vi "test tools list output schema.vi"(8 "error in (no error)":errorcluster) -> (0 "error out":errorcluster, 3 "body":string)   [LabVIEW 2020, in "MCP Server tests.lvlib"]
doc: "tools/list gives every tool with non-picture outputs an outputSchema. For fake_tool_picture_outputs it is an object schema whose properties and required list exactly count, label, mode and time, the names that tools/call returns in structuredContent, without the picture output. The property schemas are built like the input schemas, without default: time (timestamp) is a string with format date-time, mode (enum) has enum [\"slow\",\"fast\"], count is an integer with the description of its indicator. A tool without outputs (fake_tool_no_inputs_outputs) has no outputSchema. The requests are sent with the LabVIEW HTTP Client directly."
uses:
  MCP Server tests.lvlib
  76897956-0dee-4ca4-8c48-61d2eaeac07d.vi
  c19c7c96-80ec-4cdf-8c59-ab371bb35518.vi
  31ad5ed3-fed4-46a9-ac69-80efe7dec1a8.vi
  8415a791-681a-46d9-8f15-2bdb6ca1e76c.vi
  <vilib>/JDP Science/JSONtext/Next JSON Value.vi
  <vilib>/JDP Science/JSONtext/String Subset.vi
  <vilib>/JDP Science/JSONtext/Parsing/Advance past next JSON Value (inlined COPY).vi
  <vilib>/JDP Science/JSONtext/Parsing/Advance past whitespace.vi
  <vilib>/JDP Science/JSONtext/Parsing/Advance past String.vi
  <vilib>/JDP Science/JSONtext/Parsing/Advance past Number.vi
  <vilib>/JDP Science/JSONtext/Parsing/Advance past Line Ending.vi
  <vilib>/JDP Science/JSONtext/Parsing/Parse Full Path or Item Name.vi
  <vilib>/JDP Science/JSONtext/Parsing/Advance past Array.vi
  <vilib>/JDP Science/JSONtext/Parsing/Advance past Object.vi
  <vilib>/JDP Science/JSONtext/support/Error Cluster From Code.vi
  <vilib>/JDP Science/JSONtext/Offset/Find Item Locations by Path.vi
  <vilib>/JDP Science/JSONtext/JSON text to Variant.vi
  <vilib>/JDP Science/JSONtext/LVClass Serializer/JSONtext LVClass Serializer.lvclass
  <vilib>/addons/_JKI Toolkits/Caraya/classes/Test/Test.lvclass
  <vilib>/JDP Science/JSONtext/JSONtext.lvlib
  <vilib>/addons/_JKI Toolkits/Caraya/classes/Assert/Assert.lvclass
panel:
  out "lookup error":errorcluster
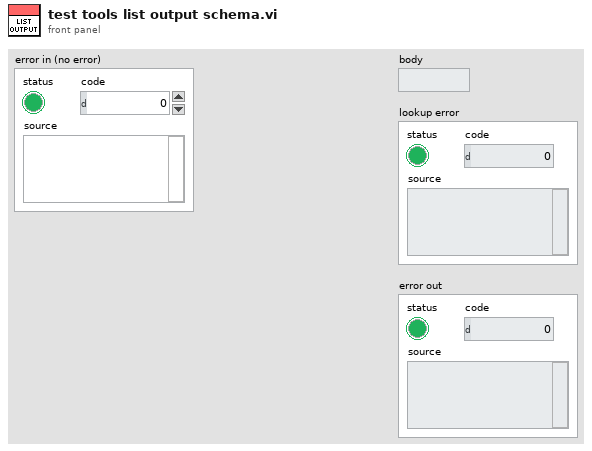
[diagram p1: front panel]
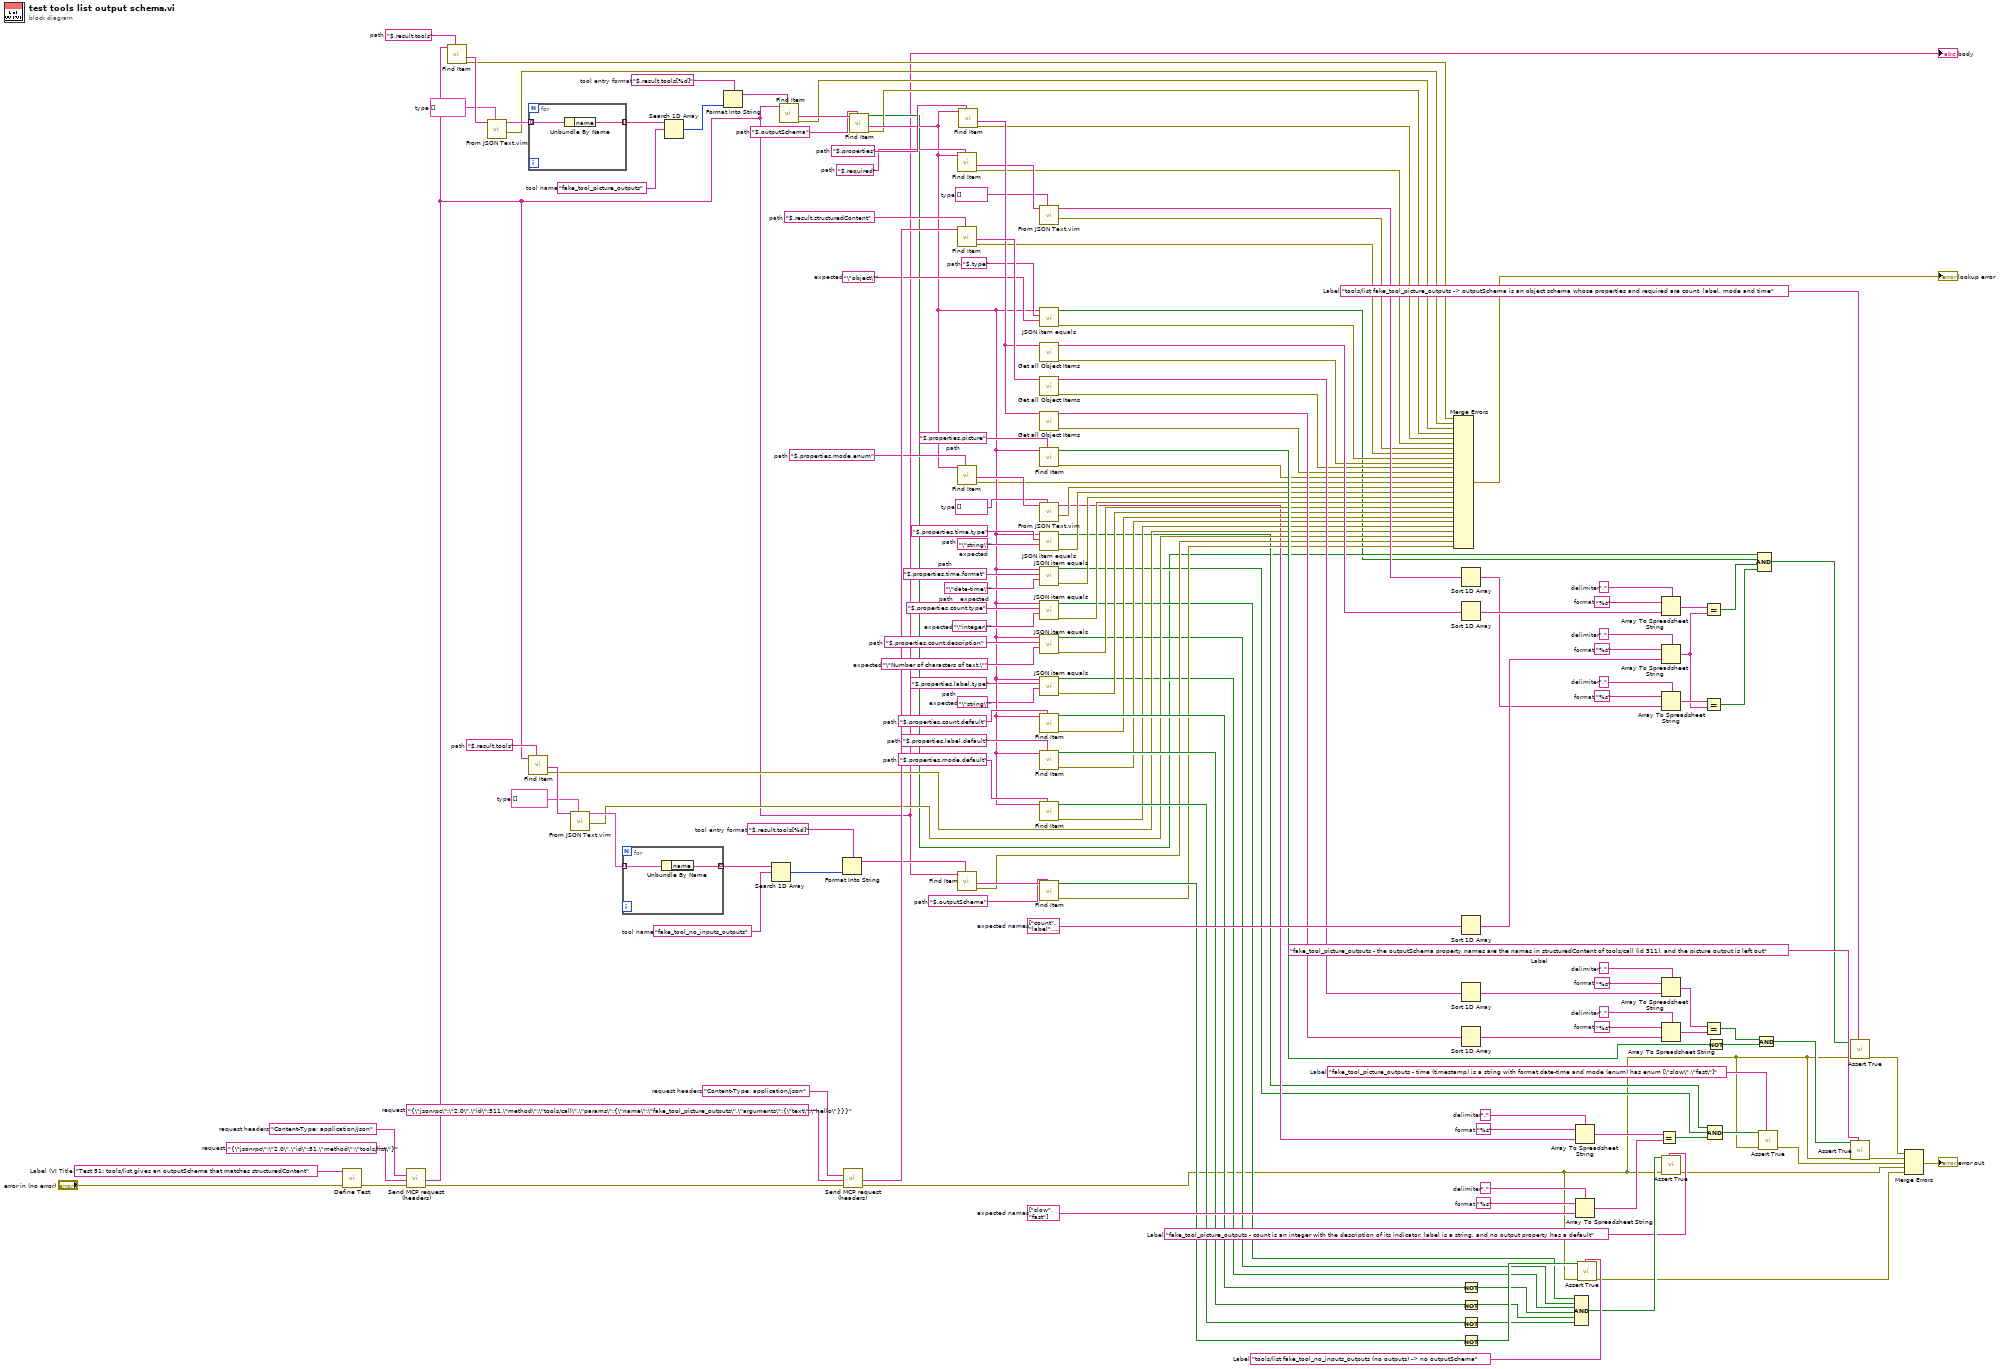
[diagram p0: block diagram]
diagram:
  w143 = "Content-Type: application/json"  # request headers
  w148 = "Content-Type: application/json"  # request headers
  w82 = "tools/list fake_tool_no_inputs_outputs (no outputs) -> no outputSchema"  # Label
  w30 = "fake_tool_picture_outputs - count is an integer with the description of its indicator, label is a string, and no output property has a default"  # Label
  w14 = "fake_tool_picture_outputs - time (timestamp) is a string with format date-time and mode (enum) has enum [\"slow\",\"fast\"]"  # Label
  w12 = "fake_tool_picture_outputs - the outputSchema property names are the names in structuredContent of tools/call (id 511), and the picture output is left out"  # Label
  w9 = "tools/list fake_tool_picture_outputs -> outputSchema is an object schema whose properties and required are count, label, mode and time"  # Label
  w114 = "$.outputSchema"  # path
  w123 = "$.result.tools[%d]"  # tool entry format
  w128 = "fake_tool_no_inputs_outputs"  # tool name
  w137 = cluster{"name":string}[] []  # type
  w144 = "$.result.tools"  # path
  w107 = "$.properties.mode.default"  # path
  w108 = "$.properties.label.default"  # path
  w109 = "$.properties.count.default"  # path
  w87 = "\"string\""  # expected
  w88 = "$.properties.label.type"  # path
  w90 = "\"Number of characters of text.\""  # expected
  w91 = "$.properties.count.description"  # path
  w92 = "\"integer\""  # expected
  w93 = "$.properties.count.type"  # path
  w152 = ","  # delimiter
  w154 = "%s"  # format
  w153 = string[] ["slow", "fast"]  # expected names
  w49 = ","  # delimiter
  w51 = "%s"  # format
  w94 = "\"date-time\""  # expected
  w95 = "$.properties.time.format"  # path
  w96 = "\"string\""  # expected
  w97 = "$.properties.time.type"  # path
  w98 = string[] []  # type
  w110 = "$.properties.mode.enum"  # path
  w111 = "$.properties.picture"  # path
  w37 = ","  # delimiter
  w39 = "%s"  # format
  w120 = ","  # delimiter
  w122 = "%s"  # format
  w34 = ","  # delimiter
  w36 = "%s"  # format
  w40 = ","  # delimiter
  w42 = "%s"  # format
  w101 = "\"object\""  # expected
  w102 = "$.type"  # path
  w149 = ","  # delimiter
  w151 = "%s"  # format
  w155 = string[] ["count", "label", "mode", "time"]  # expected names
  w135 = "$.result.structuredContent"  # path
  w103 = string[] []  # type
  w112 = "$.required"  # path
  w113 = "$.properties"  # path
  w116 = "$.outputSchema"  # path
  w125 = "$.result.tools[%d]"  # tool entry format
  w130 = "fake_tool_picture_outputs"  # tool name
  w139 = cluster{"name":string}[] []  # type
  w145 = "$.result.tools"  # path
  w142 = "{\"jsonrpc\":\"2.0\",\"id\":511,\"method\":\"tools/call\",\"params\":{\"name\":\"fake_tool_picture_outputs\",\"arguments\":{\"text\":\"hello\"}}}"  # request
  w147 = "{\"jsonrpc\":\"2.0\",\"id\":51,\"method\":\"tools/list\"}"  # request
  w157 = "Test 51: tools/list gives an outputSchema that matches structuredContent"  # Label (VI Title)
  n1 = call <vilib>:"Define Test.vi"("error in (no error)"="error in (no error)", "Label (VI Title)"=w157) -> ("error out"=w146:errorcluster)  [unwired: 8 in, 1 out]
  n2 = call "Send MCP request (headers).vi"("error in (no error)"=w146, "request"=w147, "request headers"=w148) -> ("error out"=w141:errorcluster, "response"=w3:string)  [unwired: 5 in, 2 out]
  "body" <- w3
  n3 = call <vilib>:"Find Item.vi"("$Path or Item Name"=w145, "JSON"=w3) -> ("error out"=w78:errorcluster, "<JSON>"=w140:string)  [unwired: 6 in, 2 out]
  n4 = call "From JSON Text.vim"("Data Type and Default Value"=w139, "JSON"=w140) -> ("error out"=w77:errorcluster, "Data out"=w134:cluster{"name":string}[])  [unwired: 8 in]
  n5 = for {
    tunnel: w134 -> [w159] mode=indexing
    tunnel: [w158] -> w131 mode=indexing
    n6 = Unbundle By Name(w159) -> ("name"=w158:string)
  }
  n7 = call <vilib>:"Find Item.vi"("$Path or Item Name"=w144, "JSON"=w3) -> ("error out"=w55:errorcluster, "<JSON>"=w138:string)  [unwired: 6 in, 2 out]
  n8 = call "From JSON Text.vim"("Data Type and Default Value"=w137, "JSON"=w138) -> ("error out"=w54:errorcluster, "Data out"=w133:cluster{"name":string}[])  [unwired: 8 in]
  n9 = for {
    tunnel: w133 -> [w161] mode=indexing
    tunnel: [w160] -> w129 mode=indexing
    n10 = Unbundle By Name(w161) -> ("name"=w160:string)
  }
  n11 = Search 1D Array(1D array=w131, element=w130) -> (index of element=w126:i32)  [unwired: 1 in]
  n12 = Format Into String(format string=w125, w126) -> (resulting string=w119:string)  [unwired: 2 in, 1 out]
  n13 = Search 1D Array(1D array=w129, element=w128) -> (index of element=w124:i32)  [unwired: 1 in]
  n14 = call <vilib>:"Find Item.vi"("$Path or Item Name"=w119, "JSON"=w3) -> ("error out"=w76:errorcluster, "<JSON>"=w117:string)  [unwired: 6 in, 2 out]
  n15 = Format Into String(format string=w123, w124) -> (resulting string=w118:string)  [unwired: 2 in, 1 out]
  n16 = call "Send MCP request (headers).vi"("error in (no error)"=w141, "request"=w142, "request headers"=w143) -> ("error out"=w10:errorcluster, "response"=w136:string)  [unwired: 5 in, 2 out]
  n17 = call <vilib>:"Find Item.vi"("$Path or Item Name"=w116, "JSON"=w117) -> ("error out"=w75:errorcluster, "<JSON>"=w89:string, "Found"=w19:bool)  [unwired: 6 in, 1 out]
  n18 = call <vilib>:"Find Item.vi"("$Path or Item Name"=w112, "JSON"=w89) -> ("error out"=w73:errorcluster, "<JSON>"=w104:string)  [unwired: 6 in, 2 out]
  n19 = call <vilib>:"Find Item.vi"("$Path or Item Name"=w135, "JSON"=w136) -> ("error out"=w71:errorcluster, "<JSON>"=w132:string)  [unwired: 6 in, 2 out]
  n20 = call <vilib>:"Find Item.vi"("$Path or Item Name"=w110, "JSON"=w89) -> ("error out"=w65:errorcluster, "<JSON>"=w99:string)  [unwired: 6 in, 2 out]
  n21 = call <vilib>:"Find Item.vi"("$Path or Item Name"=w118, "JSON"=w3) -> ("error out"=w53:errorcluster, "<JSON>"=w115:string)  [unwired: 6 in, 2 out]
  n22 = call <vilib>:"Find Item.vi"("$Path or Item Name"=w113, "JSON"=w89) -> ("error out"=w74:errorcluster, "<JSON>"=w105:string)  [unwired: 6 in, 2 out]
  n23 = call "From JSON Text.vim"("Data Type and Default Value"=w103, "JSON"=w104) -> ("error out"=w72:errorcluster, "Data out"=w79:string[])  [unwired: 8 in]
  n24 = call "JSON item equals.vi"("expected"=w101, "path"=w102, "JSON"=w89) -> ("error out"=w70:errorcluster, "equal?"=w18:bool)  [unwired: 6 in, 1 out]
  n25 = call <vilib>:"Get all Object Items.vi"("JSON"=w105) -> ("error out"=w69:errorcluster, "Item Names"=w81:string[])  [unwired: 7 in, 2 out]
  n26 = call <vilib>:"Get all Object Items.vi"("JSON"=w132) -> ("error out"=w68:errorcluster, "Item Names"=w127:string[])  [unwired: 7 in, 2 out]
  n27 = call <vilib>:"Get all Object Items.vi"("JSON"=w105) -> ("error out"=w67:errorcluster, "Item Names"=w80:string[])  [unwired: 7 in, 2 out]
  n28 = call <vilib>:"Find Item.vi"("$Path or Item Name"=w111, "JSON"=w89) -> ("error out"=w66:errorcluster, "Found"=w100:bool)  [unwired: 6 in, 2 out]
  n29 = call "From JSON Text.vim"("Data Type and Default Value"=w98, "JSON"=w99) -> ("error out"=w64:errorcluster, "Data out"=w50:string[])  [unwired: 8 in]
  n30 = call "JSON item equals.vi"("expected"=w96, "path"=w97, "JSON"=w89) -> ("error out"=w63:errorcluster, "equal?"=w24:bool)  [unwired: 6 in, 1 out]
  n31 = call "JSON item equals.vi"("expected"=w94, "path"=w95, "JSON"=w89) -> ("error out"=w62:errorcluster, "equal?"=w23:bool)  [unwired: 6 in, 1 out]
  n32 = call "JSON item equals.vi"("expected"=w92, "path"=w93, "JSON"=w89) -> ("error out"=w61:errorcluster, "equal?"=w48:bool)  [unwired: 6 in, 1 out]
  n33 = call "JSON item equals.vi"("expected"=w90, "path"=w91, "JSON"=w89) -> ("error out"=w60:errorcluster, "equal?"=w47:bool)  [unwired: 6 in, 1 out]
  n34 = call "JSON item equals.vi"("expected"=w87, "path"=w88, "JSON"=w89) -> ("error out"=w59:errorcluster, "equal?"=w46:bool)  [unwired: 6 in, 1 out]
  n35 = call <vilib>:"Find Item.vi"("$Path or Item Name"=w109, "JSON"=w89) -> ("error out"=w58:errorcluster, "Found"=w86:bool)  [unwired: 6 in, 2 out]
  n36 = call <vilib>:"Find Item.vi"("$Path or Item Name"=w108, "JSON"=w89) -> ("error out"=w57:errorcluster, "Found"=w85:bool)  [unwired: 6 in, 2 out]
  n37 = call <vilib>:"Find Item.vi"("$Path or Item Name"=w107, "JSON"=w89) -> ("error out"=w56:errorcluster, "Found"=w84:bool)  [unwired: 6 in, 2 out]
  n38 = call <vilib>:"Find Item.vi"("$Path or Item Name"=w114, "JSON"=w115) -> ("error out"=w52:errorcluster, "Found"=w106:bool)  [unwired: 6 in, 2 out]
  n39 = Merge Errors(w78, w77, w76, w75, w74, w73, w72, w71, w70, w69, w68, w67, w66, w65, w64, w63, w62, w61, w60, w59, w58, w57, w56, w55, w54, w53, w52) -> (→"lookup error":errorcluster)
  n40 = Sort 1D Array(array=w79) -> (sorted array=w35:string[])
  n41 = Sort 1D Array(array=w81) -> (sorted array=w41:string[])
  n42 = Sort 1D Array(array=w155) -> (sorted array=w150:string[])
  n43 = Sort 1D Array(array=w127) -> (sorted array=w121:string[])
  n44 = Sort 1D Array(array=w80) -> (sorted array=w38:string[])
  n45 = Not(x=w86) -> (.not. x?=w45:bool)
  n46 = Not(x=w85) -> (.not. x?=w44:bool)
  n47 = Not(x=w84) -> (.not. x?=w43:bool)
  n48 = Not(x=w106) -> (.not. x?=w83:bool)
  n49 = Compound Arithmetic op=AND(w48, w47, w46, w45, w44, w43) -> (w31:bool)
  n50 = Array To Spreadsheet String(delimiter (Tab)=w49, array=w50, 3:w51) -> (spreadsheet string=w33:string)
  n51 = Array To Spreadsheet String(delimiter (Tab)=w152, array=w153, 3:w154) -> (spreadsheet string=w32:string)
  n52 = call <vilib>:"Assert True.vi"("Label"=w82, "error in (no error)"=w10, "True?"=w83) -> ("error out"=w4:errorcluster)  [unwired: 7 in, 1 out]
  n53 = Equal?(x=w33, y=w32) -> (x = y?=w22:bool)
  n54 = Array To Spreadsheet String(delimiter (Tab)=w40, array=w41, 3:w42) -> (spreadsheet string=w29:string)
  n55 = Array To Spreadsheet String(delimiter (Tab)=w149, array=w150, 3:w151) -> (spreadsheet string=w25:string)
  n56 = Array To Spreadsheet String(delimiter (Tab)=w34, array=w35, 3:w36) -> (spreadsheet string=w26:string)
  n57 = Array To Spreadsheet String(delimiter (Tab)=w120, array=w121, 3:w122) -> (spreadsheet string=w28:string)
  n58 = Array To Spreadsheet String(delimiter (Tab)=w37, array=w38, 3:w39) -> (spreadsheet string=w27:string)
  n59 = call <vilib>:"Assert True.vi"("Label"=w30, "error in (no error)"=w10, "True?"=w31) -> ("error out"=w5:errorcluster)  [unwired: 7 in, 1 out]
  n60 = Equal?(x=w29, y=w25) -> (x = y?=w17:bool)
  n61 = Equal?(x=w26, y=w25) -> (x = y?=w16:bool)
  n62 = Equal?(x=w28, y=w27) -> (x = y?=w21:bool)
  n63 = Not(x=w100) -> (.not. x?=w20:bool)
  n64 = Compound Arithmetic op=AND(w24, w23, w22) -> (w15:bool)
  n65 = Compound Arithmetic op=AND(w19, w18, w17, w16) -> (w11:bool)
  n66 = call <vilib>:"Assert True.vi"("Label"=w14, "error in (no error)"=w10, "True?"=w15) -> ("error out"=w6:errorcluster)  [unwired: 7 in, 1 out]
  n67 = Compound Arithmetic op=AND(w21, w20) -> (w13:bool)
  n68 = call <vilib>:"Assert True.vi"("Label"=w9, "error in (no error)"=w10, "True?"=w11) -> ("error out"=w8:errorcluster)  [unwired: 7 in, 1 out]
  n69 = call <vilib>:"Assert True.vi"("Label"=w12, "error in (no error)"=w10, "True?"=w13) -> ("error out"=w7:errorcluster)  [unwired: 7 in, 1 out]
  n70 = Merge Errors(w8, w7, w6, w5, w4) -> (→"error out":errorcluster)
